vi "measure CE Frequency Error.vi"(8 "error in (no error)":errorcluster, 11 "SA Measurement in":refnum<class "SA Measurement.lvclass">) -> (0 "error out":errorcluster, 3 "SA Measurement out":refnum<class "SA Measurement.lvclass">)   [LabVIEW 2023, in "Spectrum Analyzer.lvlib" / "SA Measurement.lvclass"]
uses:
  SA Measurement.lvclass
  SA Measurement.lvclass/SA Measurement.ctl
  TYPE DEFINITION/Keysight 9020A/TYPE Measurement Preset.ctl
  Spectrum Analyzer.lvlib
  Interface_Spectrum/Interface_Spectrum.lvclass
  TYPE DEFINITION/TYPE RBW and VBW Select.ctl
  TYPE DEFINITION/TYPE Marker Peak Search Type.ctl
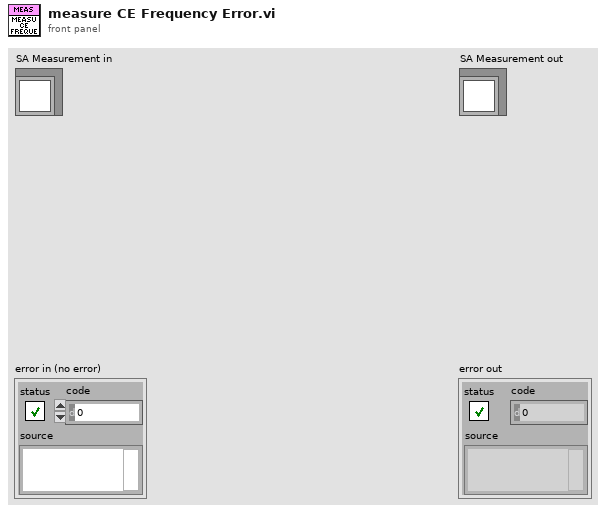
[diagram p1: front panel]
types:
  T1 = typedef "Spectrum Analyzer.lvlib/TYPE Marker Peak Search Type.ctl" = enum16{"Max", "Next Peak"}
  T2 = typedef "Spectrum Analyzer.lvlib/TYPE RBW and VBW Select.ctl" = enum16{"Res BW", "Video BW"}
  T3 = typedef "Spectrum Analyzer.lvlib/TYPE Measurement Preset.ctl" = enum16{"Sweep SA Mode", "Channel Power", "Occupied BW", "ACP", "Spurious Emission", "Spurious Emission Mask", "Burst Power (Transmit Power)"}
  T4 = typedef "Spectrum Analyzer.lvlib/TYPE Y-axis Unit.ctl" = enum16{"dBm", "dBmV", "dBuV", "dBpW", "Volt", "Ampere", "Watt"}
  T5 = typedef "Spectrum Analyzer.lvlib/TYPE Reference Level and Atten Param.ctl" = cluster{"Reference Level":dbl, "Atten":i32, "Atten Auto?":bool, "Reference Level Offset":dbl}
  T6 = typedef "Spectrum Analyzer.lvlib/TYPE Display Trace Mode Select.ctl" = enum16{"Clear Write", "Max Hold", "Min Hold", "Average", "View"}
  T7 = typedef "Spectrum Analyzer.lvlib/TYPE Detect Mode Select.ctl" = enum16{"Det Auto (Normal)", "Auto Peak", "Positive Peak", "Negative Peak", "Sample", "RMS", "Average", "Quasipeak", "CISPR Average", "RMS Average"}
  T8 = cluster{"Trace Mode":T6, "Detector Type":T7, "Detect Auto?":bool}[]
  T9 = typedef "Spectrum Analyzer.lvlib/TYPE Average Mode Select.ctl" = enum16{"Linear(Voltage Avg)", "Video(Log)", "Power"}
  T10 = typedef "Spectrum Analyzer.lvlib/TYPE Marker Value.ctl" = cluster{"X-axis":dbl, "Y-axis":dbl}
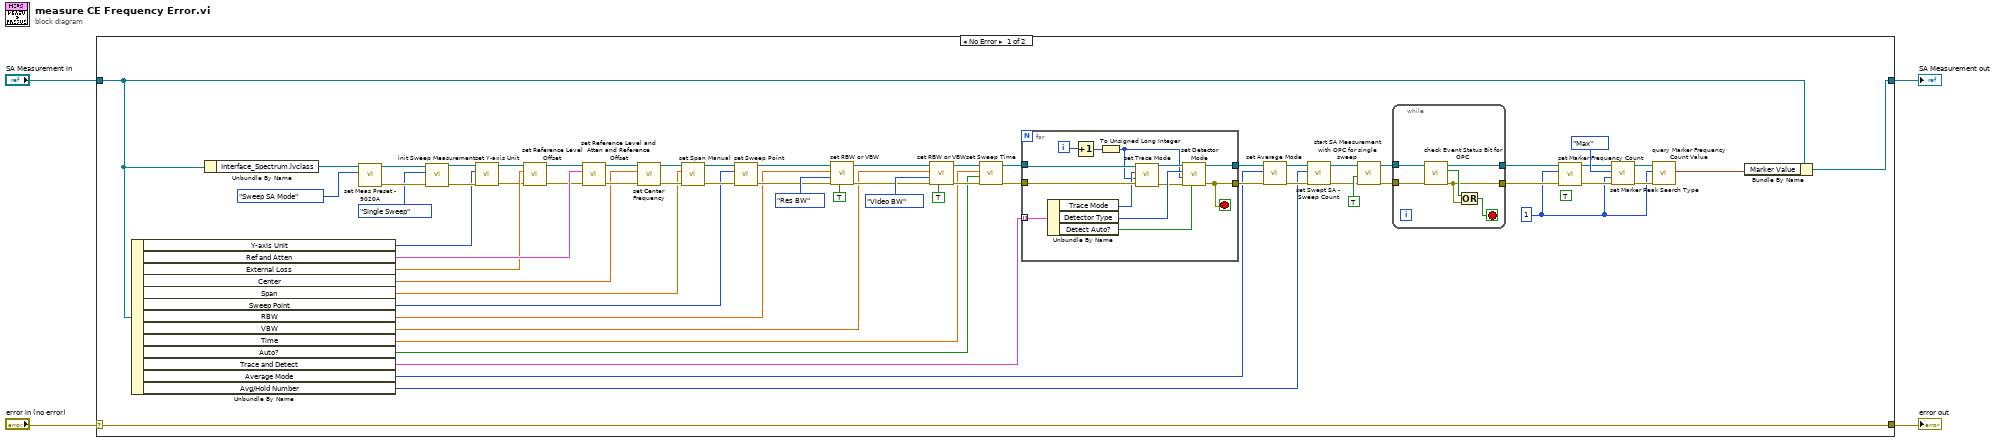
[diagram p0: block diagram]
diagram:
  n1 = case shown="No Error" "error in (no error)" {
    selector: "error in (no error)" -> [w67 w88]
    tunnel: [w67 w88] -> w3
    tunnel: [w5 w87] -> w1
    tunnel: "SA Measurement in" -> [w7 w87]
    frame No Error {
      (unwired) TRUE ("On?")
      w8 = 1 ("Index")
      n2 = Unbundle By Name(w7) -> ("Y-axis Unit"=w58:T4, "Ref and Atten"=w61:T5, "External Loss"=w57:dbl, "Center"=w48:dbl, "Span"=w47:dbl, "Sweep Point"=w44:u32, "RBW"=w35:dbl, "VBW"=w34:dbl, "Time"=w31:dbl, "Auto?"=w30:bool, "Trace and Detect"=w27:T8, "Average Mode"=w22:T9, "Avg/Hold Number"=w21:u32)
      n3 = Unbundle By Name(w7) -> ("Interface_Spectrum.lvclass"=w66:refnum<class "Interface_Spectrum.lvclass">)
      n4 = call-dynamic "set Meas Preset - 9020A.vi"("Measurement Preset"=TYPE_Measurement_Preset."Sweep SA Mode", "Interface_Spectrum in"=w66) -> ("error out"=w63:errorcluster, "Interface_Spectrum out"=w64:refnum<class "Interface_Spectrum.lvclass">)  [unwired: 8 in]
      n5 = call-dynamic "init Sweep Measurement.vi"("error in (no error)"=w63, "Sweep Measurement Mode"=enum16{"Single Sweep", "Continuous Sweep"}."Single Sweep", "Interface_Spectrum in"=w64) -> ("error out"=w59:errorcluster, "Interface_Spectrum out"=w60:refnum<class "Interface_Spectrum.lvclass">)  [unwired: 7 in]
      n6 = call-dynamic "set Y-axis Unit.vi"("error in (no error)"=w59, "Y-axis Unit"=w58, "Interface_Spectrum in"=w60) -> ("error out"=w55:errorcluster, "Interface_Spectrum out"=w56:refnum<class "Interface_Spectrum.lvclass">)  [unwired: 7 in]
      n7 = call-dynamic "set Reference Level Offset.vi"("error in (no error)"=w55, "Reference Level Offset"=w57, "Interface_Spectrum in"=w56) -> ("error out"=w53:errorcluster, "Interface_Spectrum out"=w54:refnum<class "Interface_Spectrum.lvclass">)  [unwired: 7 in]
      n8 = call-dynamic "set Reference Level and Atten and Reference Offset.vi"("error in (no error)"=w53, "Reference Level, Atten, Reference Offset"=w61, "Interface_Spectrum in"=w54) -> ("error out"=w49:errorcluster, "Interface_Spectrum out"=w50:refnum<class "Interface_Spectrum.lvclass">)  [unwired: 7 in]
      n9 = call-dynamic "set Center Frequency.vi"("error in (no error)"=w49, "Center Frequency (Hz)"=w48, "Interface_Spectrum in"=w50) -> ("error out"=w51:errorcluster, "Interface_Spectrum out"=w52:refnum<class "Interface_Spectrum.lvclass">)  [unwired: 7 in]
      n10 = call-dynamic "set Span Manual.vi"("error in (no error)"=w51, "Span (Hz)"=w47, "Interface_Spectrum in"=w52) -> ("error out"=w45:errorcluster, "Interface_Spectrum out"=w46:refnum<class "Interface_Spectrum.lvclass">)  [unwired: 7 in]
      n11 = call-dynamic "set Sweep Point.vi"("error in (no error)"=w45, "Sweep Point"=w44, "Interface_Spectrum in"=w46) -> ("error out"=w36:errorcluster, "Interface_Spectrum out"=w37:refnum<class "Interface_Spectrum.lvclass">)  [unwired: 7 in]
      n12 = call-dynamic "set RBW or VBW.vi"("BW Auto?"=TRUE, "error in (no error)"=w36, "BW Type"=TYPE_RBW_and_VBW_Select."Res BW", "BW Value (Hz)"=w35, "Interface_Spectrum in"=w37) -> ("error out"=w38:errorcluster, "Interface_Spectrum out"=w39:refnum<class "Interface_Spectrum.lvclass">)  [unwired: 5 in]
      n13 = call-dynamic "set RBW or VBW.vi"("BW Auto?"=TRUE, "error in (no error)"=w38, "BW Type"=TYPE_RBW_and_VBW_Select."Video BW", "BW Value (Hz)"=w34, "Interface_Spectrum in"=w39) -> ("error out"=w32:errorcluster, "Interface_Spectrum out"=w33:refnum<class "Interface_Spectrum.lvclass">)  [unwired: 5 in]
      n14 = call-dynamic "set Sweep Time.vi"("error in (no error)"=w32, "Sweep Time Auto?"=w30, "Sweep Time(sec)"=w31, "Interface_Spectrum in"=w33) -> ("error out"=w28:errorcluster, "Interface_Spectrum out"=w29:refnum<class "Interface_Spectrum.lvclass">)  [unwired: 6 in]
      n15 = for {
        tunnel: w29 -> [w85]
        tunnel: w28 -> [w84]
        tunnel: w27 -> [w86] mode=indexing
        tunnel: [w74] -> w23
        tunnel: [w75] -> w24
        i -> [w83]
        stop <- w74 stop-if-true
        n16 = Unbundle By Name(w86) -> ("Trace Mode"=w81:T6, "Detector Type"=w79:T7, "Detect Auto?"=w76:bool)
        n17 = Increment(x=w83) -> (x+1=w82:i32)
        n18 = To Unsigned Long Integer(number=w82) -> (unsigned 32bit integer=w77:u32)
        n19 = call-dynamic "set Trace Mode.vi"("error in (no error)"=w84, "Trace Index"=w77, "Trace Mode"=w81, "Interface_Spectrum in"=w85) -> ("error out"=w78:errorcluster, "Interface_Spectrum out"=w80:refnum<class "Interface_Spectrum.lvclass">)  [unwired: 6 in]
        n20 = call-dynamic "set Detector Mode.vi"("Detect Auto?"=w76, "error in (no error)"=w78, "Trace Index"=w77, "Detector Type"=w79, "Interface_Spectrum in"=w80) -> ("error out"=w74:errorcluster, "Interface_Spectrum out"=w75:refnum<class "Interface_Spectrum.lvclass">)  [unwired: 5 in]
      }
      n21 = call-dynamic "set Average Mode.vi"("error in (no error)"=w23, "Average Mode"=w22, "Interface_Spectrum in"=w24) -> ("error out"=w25:errorcluster, "Interface_Spectrum out"=w26:refnum<class "Interface_Spectrum.lvclass">)  [unwired: 7 in]
      n22 = call-dynamic "set Swept SA - Sweep Count.vi"("error in (no error)"=w25, "Sweep Count"=w21, "Interface_Spectrum in"=w26) -> ("error out"=w15:errorcluster, "Interface_Spectrum out"=w16:refnum<class "Interface_Spectrum.lvclass">)  [unwired: 7 in]
      n23 = call-dynamic "start SA Measurement with OPC for single sweep.vi"("error in (no error)"=w15, "with OPC?"=TRUE, "Interface_Spectrum in"=w16) -> ("error out"=w18:errorcluster, "Interface_Spectrum out"=w19:refnum<class "Interface_Spectrum.lvclass">)  [unwired: 7 in]
      n24 = while {
        tunnel: w19 -> [w73]
        tunnel: w18 -> [w72]
        tunnel: [w69] -> w13
        tunnel: [w68] -> w14
        stop <- w70 stop-if-true
        n25 = call-dynamic "check Event Status Bit for OPC.vi"("error in (no error)"=w72, "Interface_Spectrum in"=w73) -> ("error out"=w69:errorcluster, "OPC Bit Changed?"=w71:bool, "Interface_Spectrum out"=w68:refnum<class "Interface_Spectrum.lvclass">)  [unwired: 7 in]
        n26 = Or(x=w71, y=w69) -> (x .or. y?=w70:bool)
      }
      n27 = call-dynamic "set Marker Frequency Count.vi"("error in (no error)"=w13, "Index"=w8, "Interface_Spectrum in"=w14) -> ("error out"=w11:errorcluster, "Interface_Spectrum out"=w12:refnum<class "Interface_Spectrum.lvclass">)  [unwired: 7 in]
      n28 = call-dynamic "set Marker Peak Search Type.vi"("error in (no error)"=w11, "Marker Index"=w8, "Peak Search Type"=TYPE_Marker_Peak_Search_Type."Max", "Interface_Spectrum in"=w12) -> ("error out"=w9:errorcluster, "Interface_Spectrum out"=w10:refnum<class "Interface_Spectrum.lvclass">)  [unwired: 6 in]
      n29 = call-dynamic "query Marker Frequency Count Value.vi"("error in (no error)"=w9, "Marker Index"=w8, "Interface_Spectrum in"=w10) -> ("Marker Value"=w6:T10)  [unwired: 6 in, 2 out]
      n30 = Bundle By Name(cluster=w7, "Marker Value"=w6) -> (w5:refnum<class "SA Measurement.lvclass">)
    }
    frame Error {
    }
  }
  "error out" <- w3
  "SA Measurement out" <- w1
